vi "trunGyro.vi"() -> ()   [LabVIEW 2019]
uses:
  <vilib>/Platform/TimedLoop/XDataNode/timing_clust.ctl
  <vilib>/Platform/TimedLoop/XDataNode/nitl_modes.ctl
  <vilib>/Platform/TimedLoop/XDataNode/wakeup.ctl
  <vilib>/Utility/error.llb/Error Cluster From Error Code.vi
  <vilib>/myRIO/Common/Instrument Driver Framework/myRIO v1.0/I2C/vis/myRIO v1.0 Write I2C.vi
  <vilib>/myRIO/Common/Instrument Driver Framework/myRIO v1.0/I2C/vis/myRIO v1.0 Read I2C.vi
  <vilib>/platform/TimedLoop/XDataNode/XDataNode.xnode
  <vilib>/Platform/TimedLoop/XDataNode/XDNodeRunTimeDep.lvlib
  <vilib>/myRIO/Instrument Drivers/Onboard IO/I2C/I2C.lvlib
panel:
  in  "旋轉":dbl=90.0 format="%#_13g"
  out "Array":dbl[][](array[numeric])
  out "旋轉偏移角度":dbl[](array[numeric])
  out "Bytes Read":u8[](array[numeric])=[127, 22, 216, 255, 15, 0]
  out "x/y":cluster{"Yaw":dbl, "Roll":dbl, "Pitch":dbl}={"Yaw"=359.9375, "Roll"=-2.5, "Pitch"=0.9375}
  in  "reset":bool
  out "現偏移角度":dbl=-0.0625
  out "可執行":bool=TRUE
  in  "Acc":dbl=0.002 format="%#_13g"
  in  "Max S":dbl=5.0 format="%#_13g"
  out "error out":errorcluster
  in  "value":dbl=68.0 format="%#_13g"
  out "Speed":dbl[](graph)
  out "Position":dbl[](graph)
  in  "error in (no error)":errorcluster
  out "output":dbl[](array[numeric])=[-0.3337499999997817, 0.6662500000002183]
  out "ENC":dbl[](array[numeric])=[10516.0, -10565.0]
  out "x .and. y?":bool=TRUE
  out "Waveform Chart":dbl[](graph)
  out "x+y":dbl[](array[numeric])=[-24.333749999999693, -24.333749999999693]
  in  "Stop Button":bool
  in  "PID gains":T1={"proportional gain (Kc)"=1.0, "integral time (Ti, min)"=0.0, "derivative time (Td, min)"=0.003} {"derivative time (Td, min)" format="%.3f"; "integral time (Ti, min)" format="%.3f"; "proportional gain (Kc)" format="%.3f"}
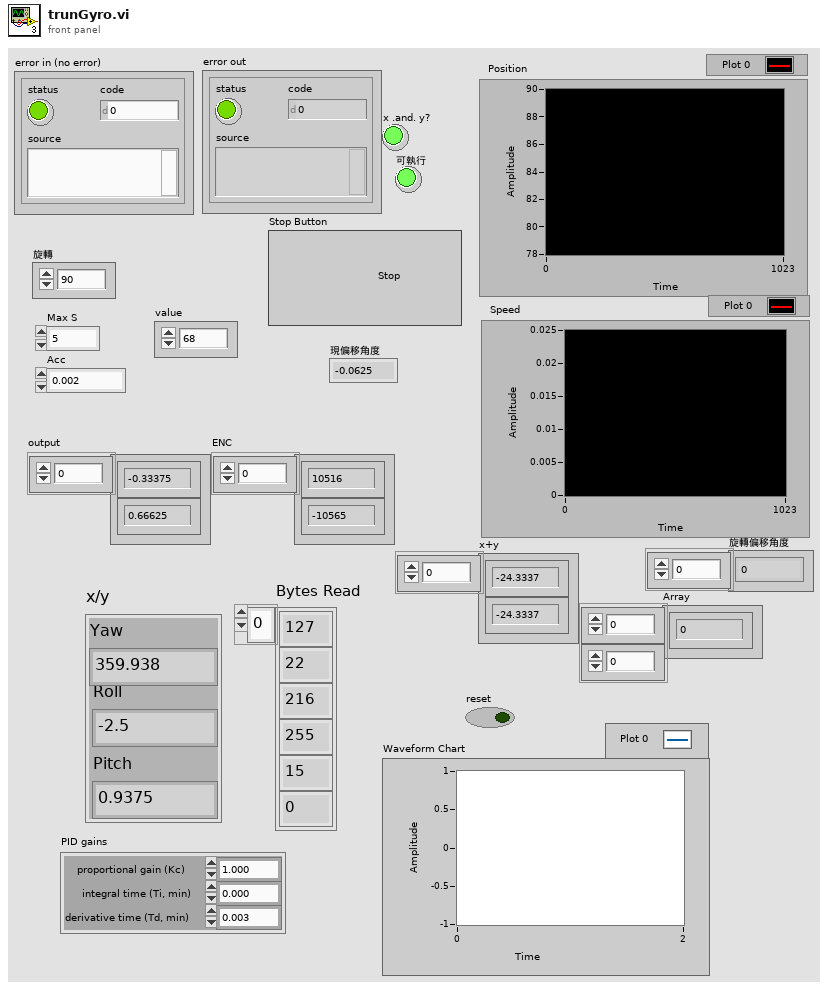
[diagram p1: front panel]
types:
  T1 = cluster{"proportional gain (Kc)":dbl, "integral time (Ti, min)":dbl, "derivative time (Td, min)":dbl}
  T2 = typedef "I2C.lvlib/I2C Reference.ctl" = cluster{"myRIO Reference":T3, "I2C Channels Enum":T7, "I2C Configuration":T8}
  T3 = typedef "myRIO Generic Hardware Reference.ctl" = cluster{"myRIO Model":T4, "myRIO Hardware Reference":T5}
  T4 = typedef "Hardware Version Enum.ctl" = enum16{"Unknown", "myRIO-1900", "myRIO-1950", "roboRIO", "NI ELVIS RIO CM", "ELVIS III"}
  T5 = typedef "myRIO v1.0 Reference.ctl" = cluster{"Generic FPGA Reference":T6, "Allow multiple opens":bool}
  T6 = typedef "Generic FPGA Reference.ctl" = refnum<k20>
  T7 = typedef "I2C Channels Enum.ctl" = enum16{"Not Connected", "A/I2C", "B/I2C", "I2C/I2C"}
  T8 = typedef "I2C.lvlib/I2C Configuration.ctl" = cluster{"I2C Transfer Rate":T9}
  T9 = typedef "I2C.lvlib/I2C Transfer Rate.ctl" = enum16{"Standard mode (100 kbps)", "Fast mode (400 kbps)"}
  T10 = typedef "XDNodeRunTimeDep.lvlib/timing_clust.ctl" = cluster{"Expected End [f-1]":u64, "Actual End [f-1]":u64, "Finished Late? [f-1]":bool, "Expected End [i-1]":u64, "Actual End [i-1]":u64, "Finished Late? [i-1]":bool, "Expected Start [i]":u64, "Actual Start [i]":u64, "Expected Start [f]":u64, "Actual Start [f]":u64, "Source Name":string, "Structure Name":string, "Period":i64, "Deadline":i64, "Offset":i64, "Start":i64, "Priority":i32, "Timeout":i32, "Mode":T11, "Wakeup Reason":T12, "Error":errorcluster, "Source Type":string, "Secondary Source Type":string, "Global End Time":u64, "Global Start Time":u64, "Frame Duration":u64, "Iteration Duration":u64, "Assigned CPU":i32, "I/O Scan Engine Mode":u32}
  T11 = typedef "XDNodeRunTimeDep.lvlib/nitl_modes.ctl" = enum32{"No Change", "Process missed periods, maintain original phase", "Discard missed periods, maintain original phase", "Process missed periods, ignore original phase", "Discard missed periods, ignore original phase"}
  T12 = typedef "XDNodeRunTimeDep.lvlib/wakeup.ctl" = enum32{"Normal", "Aborted", "Asynchronous wakeup", "Timing source error", "Timed loop error", "Timeout"}
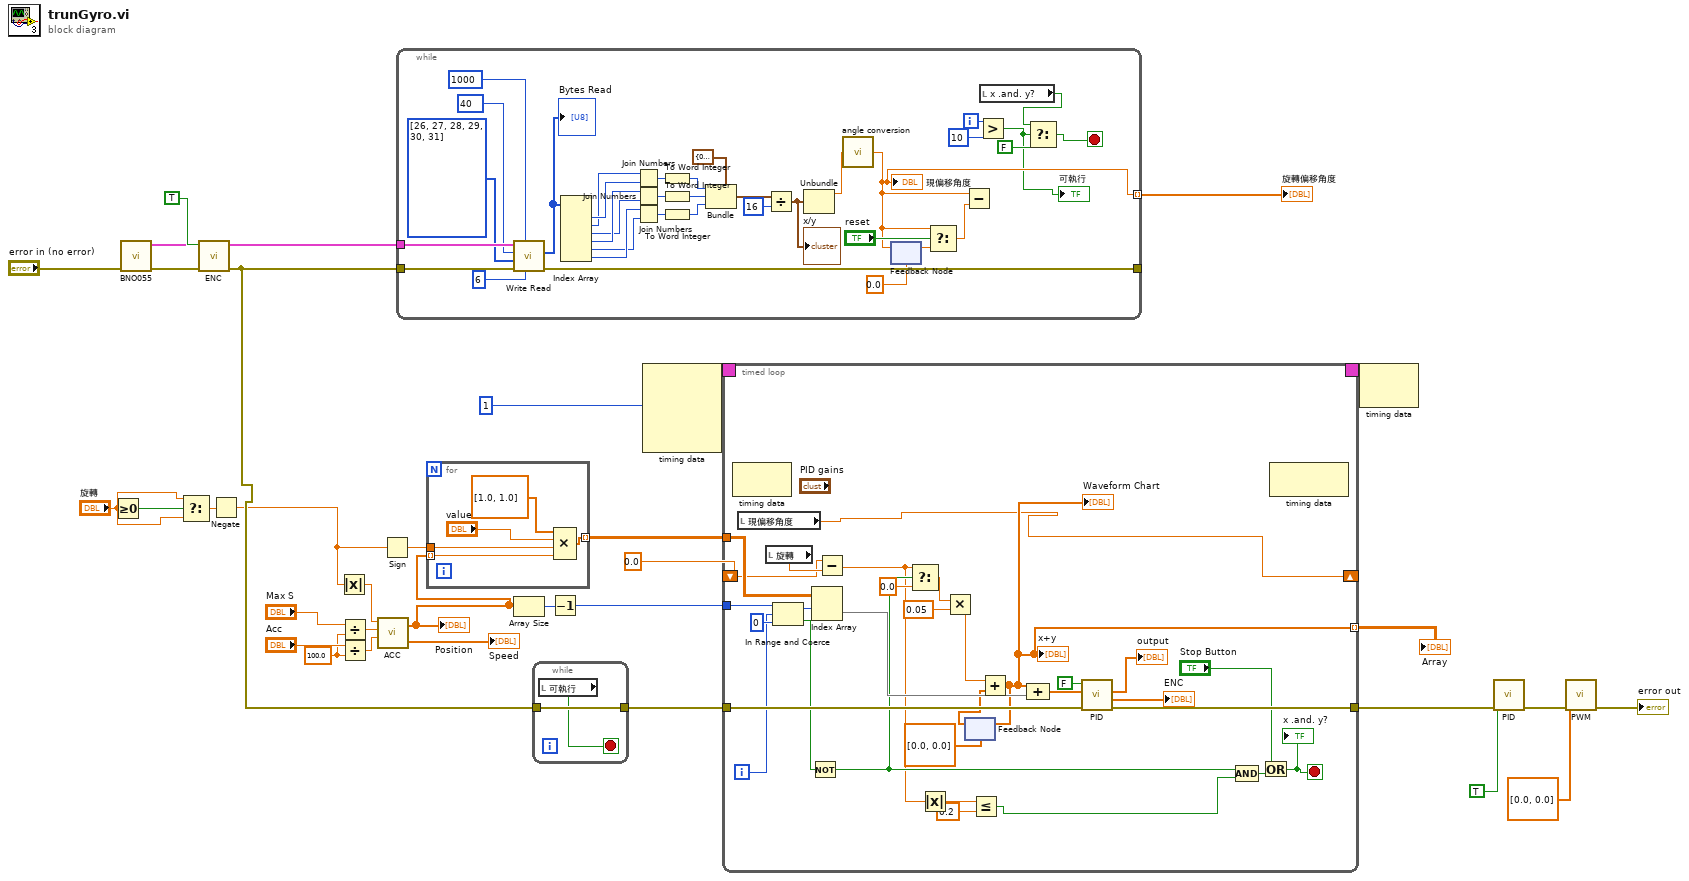
[diagram p0: block diagram]
diagram:
  w17 = 100.0 ("y")
  n1 = Greater Or Equal To 0?(x="旋轉") -> (x >= 0?=w6:bool)
  n2 = call "BNO055.vi"("error in (no error)"="error in (no error)") -> ("error out"=w7:errorcluster, "I2C Ref Out"=w14:T2)  [unwired: 9 in]
  n3 = Select(t="旋轉", s=w6, f="旋轉") -> (s? t:f=w5:dbl)
  n4 = call "ENC.vi"("error in (no error)"=w7, "Reset"=TRUE) -> ("error out"=w4:errorcluster)  [unwired: 6 in, 3 out]
  n5 = Negate(x=w5) -> (-x=w3:dbl)
  n6 = Absolute Value(x=w3) -> (abs(x)=w13:dbl)
  n7 = Divide(x="Max S", y=w17) -> (x/y=w20:dbl)
  n8 = Divide(x="Acc", y=w17) -> (x/y=w18:dbl)
  n9 = call "ACC.vi"("Acc"=w18, "Max S"=w20, "Target"=w13) -> ("Speed"=→"Speed":dbl[], "Position"=w2:dbl[])  [unwired: 1 in]
  "Position" <- w2
  n10 = Sign(1:w3) -> (0:w23:dbl)
  n11 = while {
    tunnel: w4 -> [w69]
    tunnel: w14 -> [w68]
    tunnel: [w44] -> _
    tunnel: [w36] -> w12 mode=indexing
    i -> [w35]
    stop <- w37 stop-if-true
    n12 = call <vilib>:"Write Read.vi"("Byte Count"=u32 6, "Timeout ms (1000)"=1000, "error in (no error)"=w69, "Bytes to Write"=i32[] [26, 27, 28, 29, 30, 31], "Slave Address (7-bit)"=40, "I2C Ref In"=w68) -> ("error out"=w44:errorcluster, "Bytes Read"=w63:u8[])  [unwired: 2 in, 1 out]
    "Bytes Read" <- w63
    n13 = Index Array(array=w63) -> (element #1=w51:u8, element #2=w47:u8, element #3=w57:u8, element #4=w58:u8, element #5=w55:u8, element #6=w56:u8)  [unwired: 6 in]
    n14 = Join Numbers(hi=w47, lo=w51) -> ((hi.lo)=w54:u16)
    n15 = Join Numbers(hi=w58, lo=w57) -> ((hi.lo)=w53:u16)
    n16 = Join Numbers(hi=w56, lo=w55) -> ((hi.lo)=w52:u16)
    n17 = To Word Integer(number=w54) -> (16bit integer=w48:i16)
    n18 = To Word Integer(number=w53) -> (16bit integer=w62:i16)
    n19 = To Word Integer(number=w52) -> (16bit integer=w61:i16)
    n20 = Bundle(cluster=cluster{"Yaw":i16, "Roll":i16, "Pitch":i16} {"Yaw"=0, "Roll"=0, "Pitch"=0}, "Yaw"=w48, "Roll"=w62, "Pitch"=w61) -> (w60:cluster{"Yaw":i16, "Roll":i16, "Pitch":i16})
    n21 = Divide(x=w60, y=u32 16 ("Byte Count")) -> (x/y=w49:cluster{"Yaw":dbl, "Roll":dbl, "Pitch":dbl})
    "x/y" <- w49
    n22 = Unbundle(w49) -> ("Yaw"=w41:dbl)  [unwired: 2 out]
    n23 = call "angle conversion.vi"("Numeric Control"=w41) -> ("x+y"=w36:dbl)
    "現偏移角度" <- w36
    n24 = feedback-in #1(w36) -> ()
    n25 = feedback #1(0.0) -> (w43:dbl)
    n26 = Select(t=w36, s="reset", f=w43) -> (s? t:f=w45:dbl)
    n27 = Subtract(x=w36, y=w45) -> ()  [unwired: 1 out]
    n28 = Greater?(x=w35, y=10) -> (0:w34:bool)
    "可執行" <- w34
    n29 = local read "x .and. y?"() -> (w39:bool)
    n30 = Select(t=w39, s=w34, f=FALSE) -> (s? t:f=w37:bool)
  }
  "旋轉偏移角度" <- w12
  n31 = for {
    tunnel: w2 -> [w72] mode=indexing
    tunnel: [w71] -> w27 mode=indexing
    tunnel: w23 -> [w70]
    n32 = Compound Arithmetic op=MULTIPLY(dbl[] [1.0, 1.0], "value", w70, w72) -> (w71:dbl[])
  }
  n33 = Array Size(array=w2) -> (size(s)=w29:i32)
  n34 = while {
    tunnel: [w76] -> w10
    tunnel: w4 -> [w76]
    stop <- w75 stop-if-true
    n35 = local read "可執行"() -> (w75:bool)
  }
  n36 = Decrement(x=w29) -> (x-1=w28:i32)
  n37 = node-c288(i64 1 ("Period")) -> (w33:T10)  [unwired: 3 in]
  n38 = timed-loop {
    timing: w33 -> [_]
    timing-out: [_] -> w32
    tunnel: w10 -> [w107]
    tunnel: w28 -> [w105]
    tunnel: w27 -> [w103]
    tunnel: [w100] -> w25
    shift-right: [w88] -> _
    shift-left: 0.0 ("現偏移角度") -> [w80]
    tunnel: [w89] -> w9 mode=indexing
    i -> [w96]
    stop <- w92 stop-if-true
    n39 = node-c288() -> ()  [unwired: 1 in, 1 out]
    n40 = local read "現偏移角度"() -> (w88:dbl)
    n41 = local read "旋轉"() -> (w81:dbl)
    n42 = In Range and Coerce(upper limit=w105, x=w96, lower limit=0) -> (coerced(x)=w102:i32, In Range?=w101:bool)
    n43 = Not(x=w101) -> (.not. x?=w87:bool)
    n44 = Index Array(array=w103, index (row)=w102) -> (element=w97:dbl[])  [unwired: 1 in]
    n45 = Subtract(x=w80, y=w81) -> (x-y=w82:dbl)
    n46 = Select(t=w82, s=w87, f=0.0) -> (s? t:f=w79:dbl)
    n47 = Absolute Value(x=w82) -> (abs(x)=w85:dbl)
    n48 = Multiply(x=w79, y=0.05) -> (x*y=w78:dbl)
    n49 = feedback #2(dbl[] [0.0, 0.0]) -> (w94:dbl[])
    n50 = Less Or Equal?(x=w85, y=0.2) -> (x <= y?=w84:bool)
    n51 = Add(x=w78, y=w94) -> (x+y=w89:dbl[])
    "Waveform Chart" <- w89
    "x+y" <- w89
    n52 = feedback-in #2(w89) -> ()
    n53 = Compound Arithmetic op=ADD(w89, w97) -> (w98:dbl[])
    n54 = call "PID.vi"("error in (no error)"=w107, "目標"=w98, "Reset"=FALSE) -> ("error out"=w100:errorcluster, "ENC"=→"ENC":dbl[], "output"=→"output":dbl[])  [unwired: 4 in, 2 out]
    n55 = Compound Arithmetic op=AND(w87, w84) -> (w91:bool)
    n56 = Or(x="Stop Button", y=w91) -> (x .or. y?=w92:bool)
    "x .and. y?" <- w92
    n57 = node-c288() -> ()  [unwired: 1 in, 1 out]
  }
  "Array" <- w9
  n58 = node-c288(w32) -> ()  [unwired: 1 out]
  n59 = call "PID.vi"("error in (no error)"=w25, "Reset"=TRUE ("Reset Counter")) -> ("error out"=w15:errorcluster)  [unwired: 5 in, 4 out]
  n60 = call "PWM.vi"("error in (no error)"=w15, "power"=dbl[] [0.0, 0.0]) -> ("error out"=→"error out":errorcluster)  [unwired: 9 in]
